vi "UndoEngine.vi"(0 "Reference In":refnum<class "Graph.lvclass">, 1 "Action":enum16{"TakeSnapshot", "Undo", "Redo"}(ring), 2 "Reset":bool, 3 "graphics":refnum<class "Graphics.lvclass">, 4 "grid":refnum<class "Grid.lvclass">, 5 "error in (no error)":errorcluster, 6 "menu":refnum<k9>, 8 "UndoLevels(ignoredIfNotWired)":i32=-1) -> (14 "Reference Out":refnum<class "Graph.lvclass">, 19 "error out":errorcluster)   [LabVIEW 2020, in "Graph.lvclass"]
doc: "Save to File"
uses:
  <resource>/Framework/Providers/Open_GDS/UML/Graph_class/Graph.lvclass
  <resource>/Framework/Providers/Open_GDS/UML/Grid_class/Grid.lvclass
  <resource>/Framework/Providers/Open_GDS/UML/Graphics_class/Graphics.lvclass
  <resource>/Framework/Providers/Open_GDS/UML/UMLEditor/UMLEditor_DiagramType.ctl
  <resource>/Framework/Providers/Open_GDS/UML/AbstractNode_class/AbstractNode.lvclass
  <resource>/Framework/Providers/Open_GDS/UML/AbstractEdge_class/AbstractEdge.lvclass
  <resource>/Framework/Providers/Open_GDS/UML/General/Rectangle/Rectangle Rectangle2D.ctl
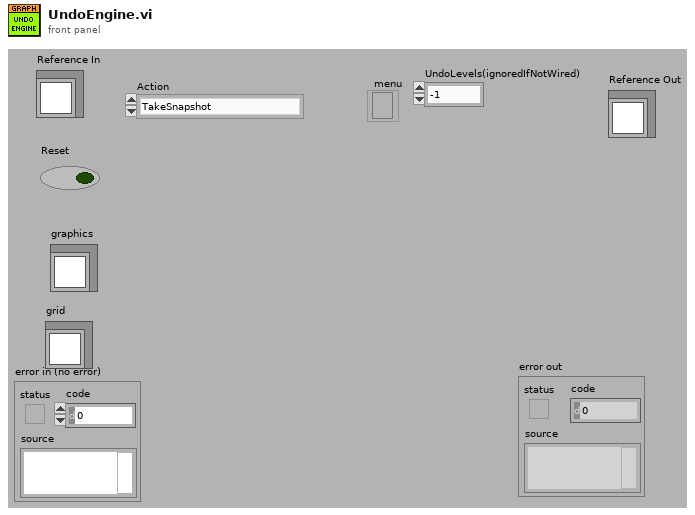
[diagram p1: front panel]
types:
  T1 = cluster{"DiagramData":string, "nodeInfo":cluster{"NodeType":string[], "ParentIndex":i32[], "ChildernIndexies":cluster{i32[]}[], "FlattenData":string[]}, "edgeInfo":cluster{"EdgeType":string[], "StartNodeIndex":i32[], "EndNodeIndex":i32[], "FlattenData":string[]}}
  T2 = cluster{"nodeInfo":cluster{"NodeType":string[], "ParentIndex":i32[], "ChildernIndexies":cluster{i32[]}[], "FlattenData":string[]}, "edgeInfo":cluster{"EdgeType":string[], "StartNodeIndex":i32[], "EndNodeIndex":i32[], "FlattenData":string[]}, "Succeeded":bool, "DiagramData":string}
  T3 = typedef "UMLEditor_DiagramType.ctl" = string
  T4 = typedef "Rectangle Rectangle2D.ctl" = cluster{"x":dbl, "y":dbl, "width":dbl, "height":dbl}
  T5 = cluster{"graph":refnum<class "Graph.lvclass">, "succeeded":bool, "diagramType":T3, "nodeInfo":cluster{"NodeType":string[], "ParentIndex":i32[], "ChildernIndexies":cluster{i32[]}[], "FlattenData":string[]}, "edgeInfo":cluster{"EdgeType":string[], "StartNodeIndex":i32[], "EndNodeIndex":i32[], "FlattenData":string[]}, "nodes":refnum<class "AbstractNode.lvclass">[], "edges":refnum<class "AbstractEdge.lvclass">[], "DiagramData":string, "bounds":T4}
  T6 = cluster{"DiagramData":string, "nodeInfo":cluster{"NodeType":string[], "ParentIndex":i32[], "ChildernIndexies":cluster{i32[]}[], "FlattenData":string[]}, "edgeInfo":cluster{"EdgeType":string[], "StartNodeIndex":i32[], "EndNodeIndex":i32[], "FlattenData":string[]}}[]
  T7 = typedef "Graph.lvclass/ObjectAttributes.ctl" = cluster{"nodes":refnum<class "AbstractNode.lvclass">[], "edges":refnum<class "AbstractEdge.lvclass">[], "nodesToBeRemoved":refnum<class "AbstractNode.lvclass">[], "edgesToBeRemoved":refnum<class "AbstractEdge.lvclass">[], "needsLayout":bool, "LayoutNodes":refnum<class "AbstractNode.lvclass">[]}
  T8 = cluster{"children":refnum<class "AbstractNode.lvclass">[]}
  T9 = cluster{"NodeType":string[], "ParentIndex":i32[], "ChildernIndexies":cluster{i32[]}[], "FlattenData":string[]}
  T10 = cluster{"EdgeType":string[], "StartNodeIndex":i32[], "EndNodeIndex":i32[], "FlattenData":string[]}
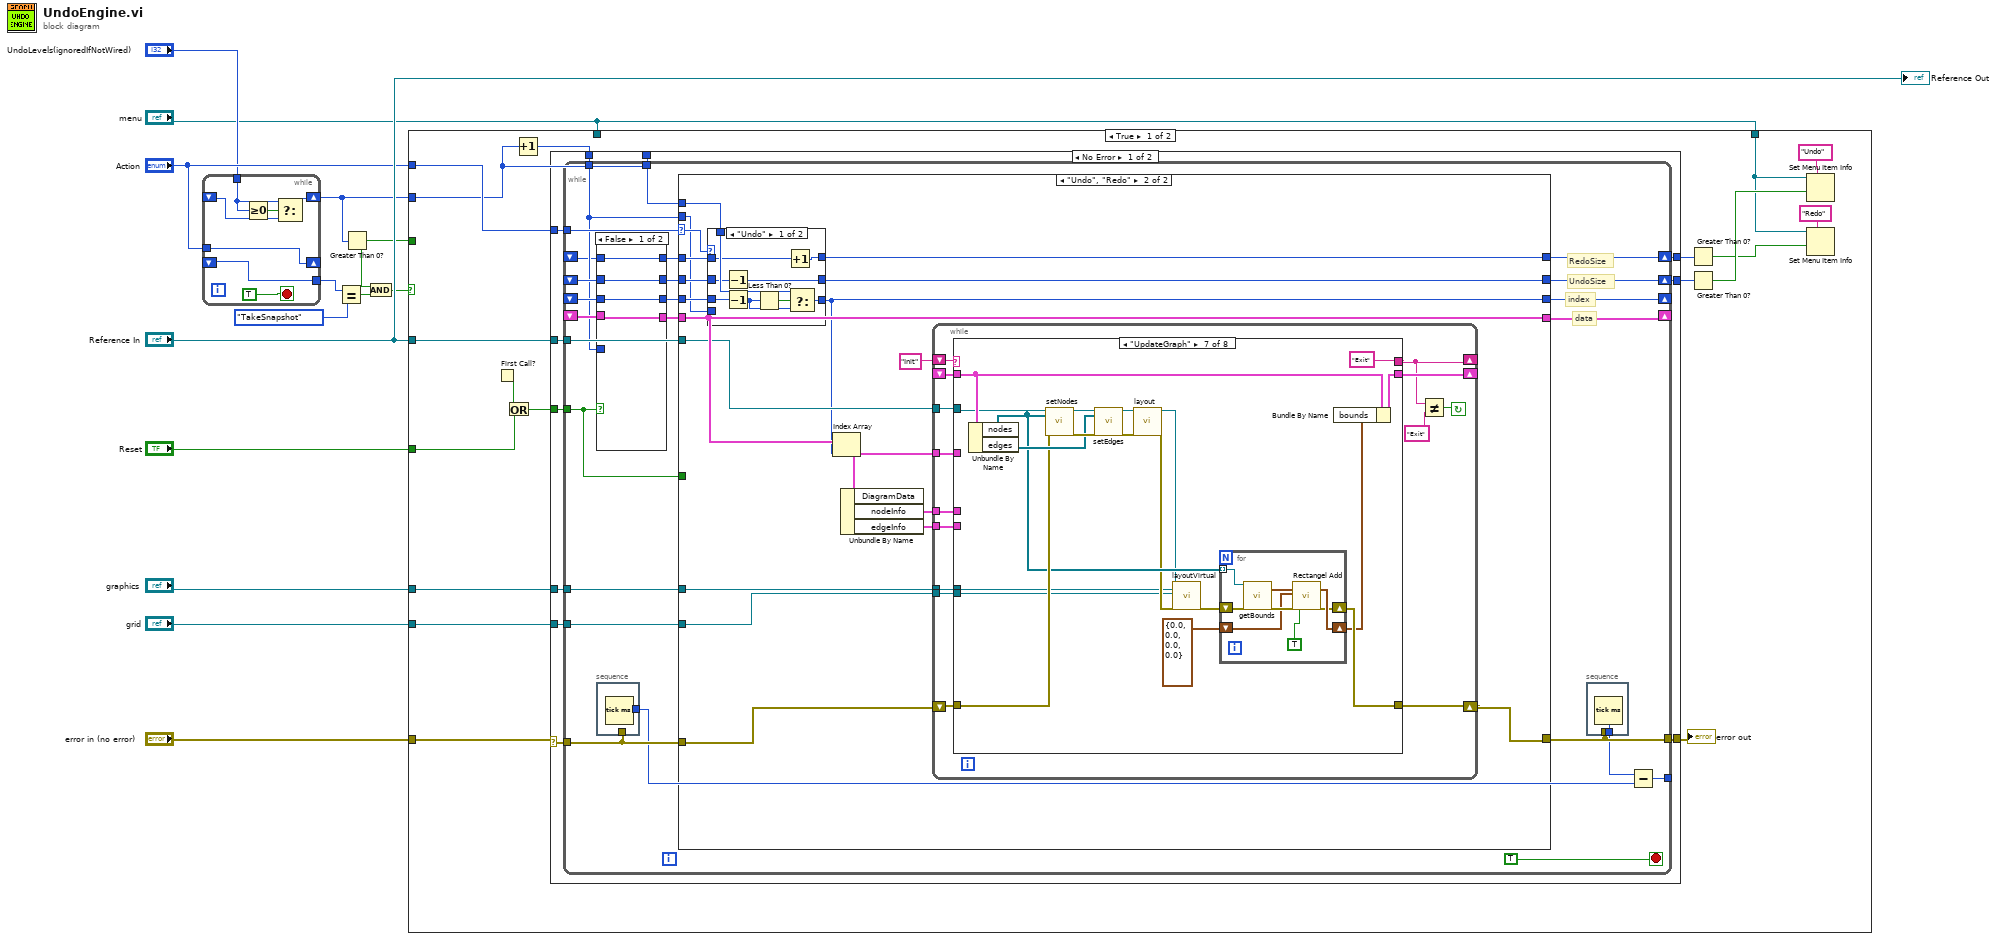
[diagram p0: block diagram]
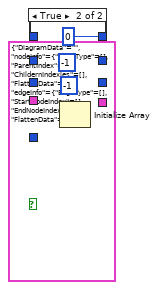
[diagram p2: hidden frame]
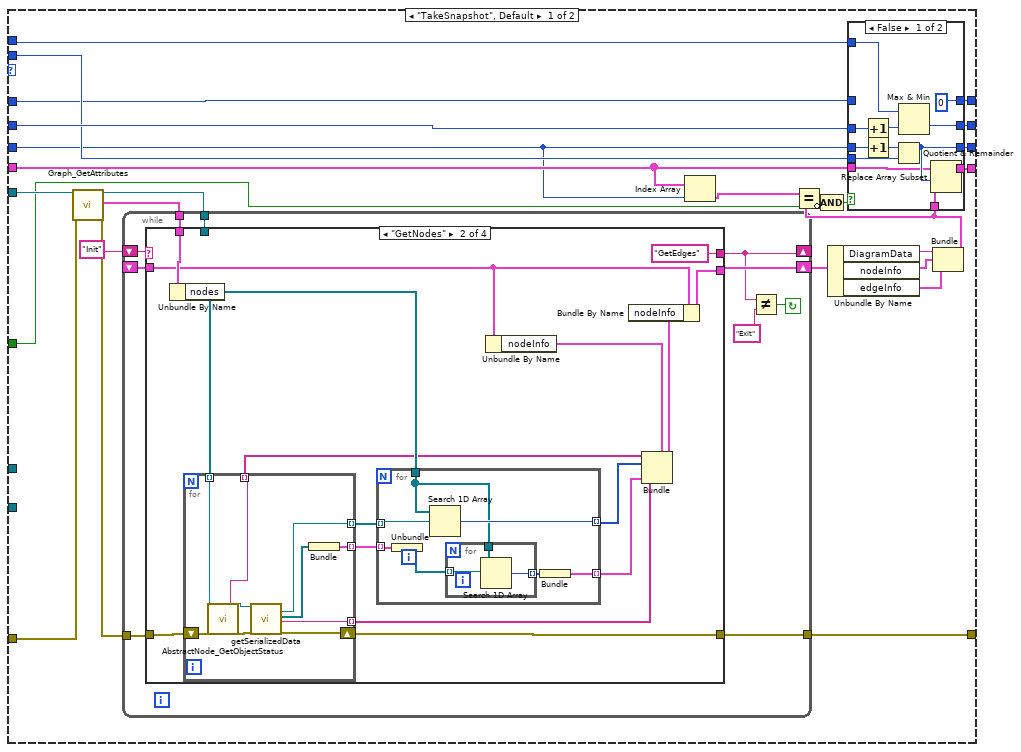
[diagram p3: hidden frame]
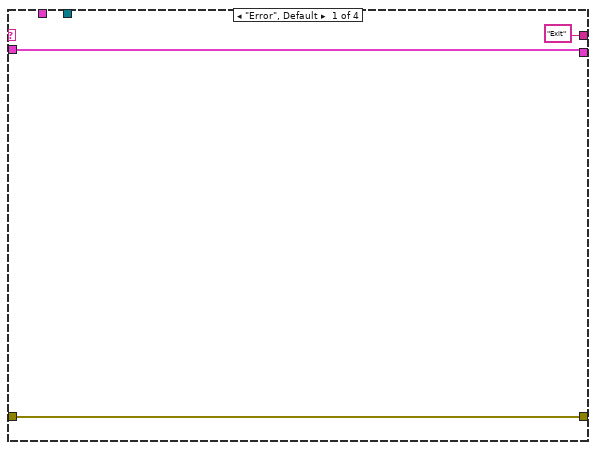
[diagram p5: hidden frame]
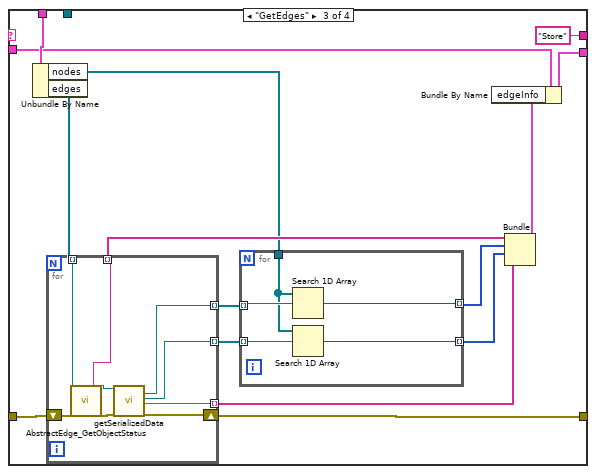
[diagram p6: hidden frame]
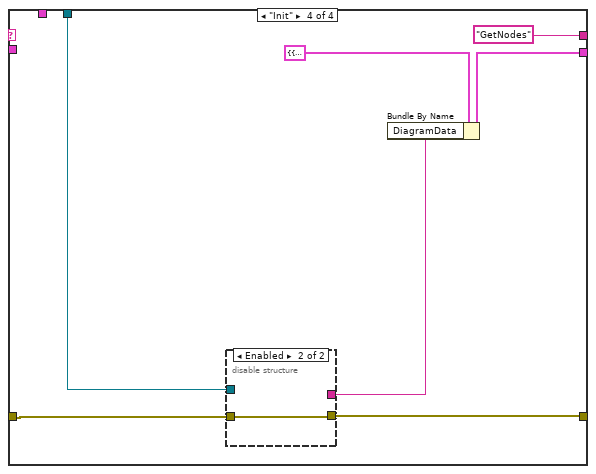
[diagram p7: hidden frame]
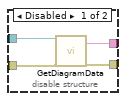
[diagram p8: hidden frame]
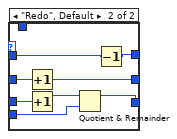
[diagram p9: hidden frame]
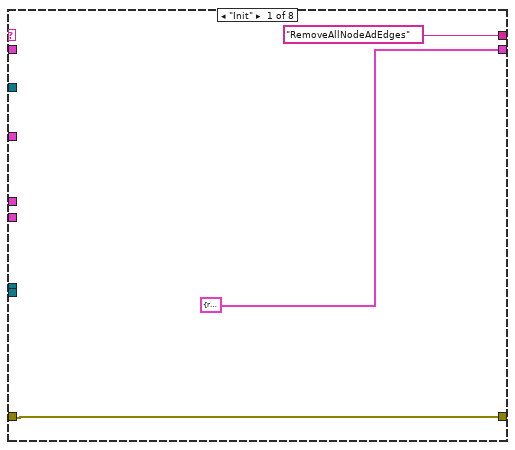
[diagram p10: hidden frame]
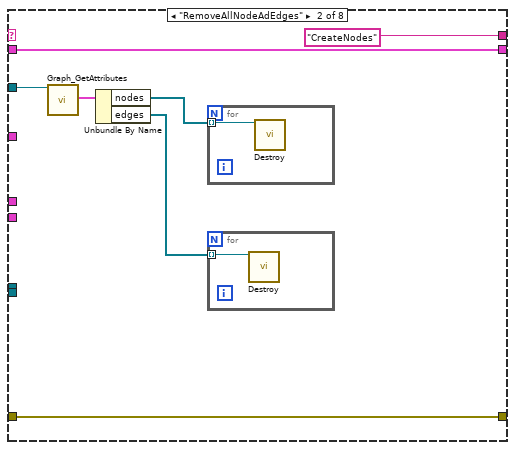
[diagram p11: hidden frame]
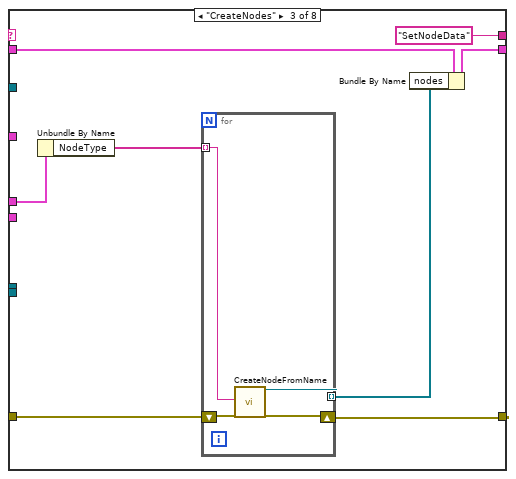
[diagram p12: hidden frame]
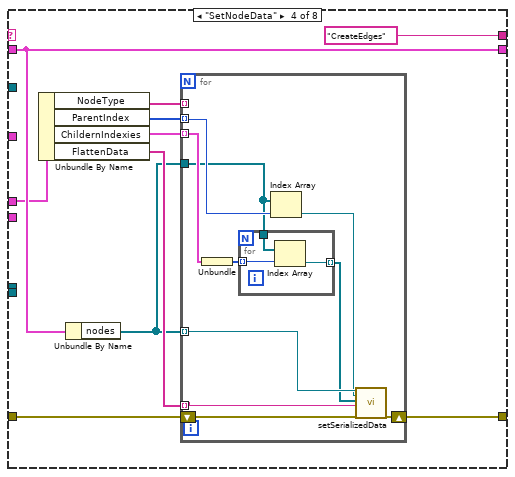
[diagram p13: hidden frame]
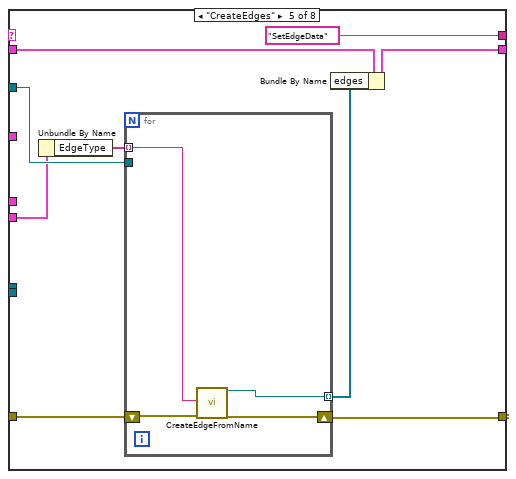
[diagram p14: hidden frame]
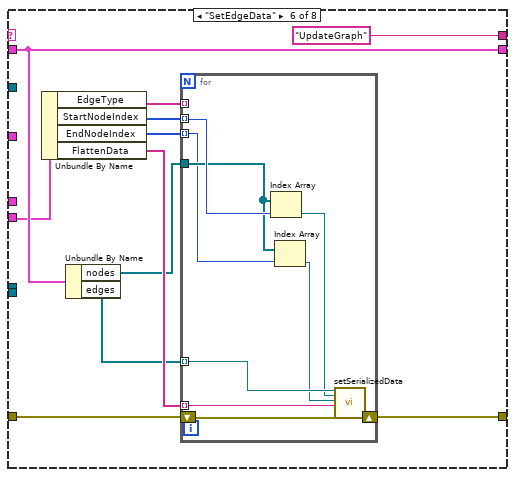
[diagram p15: hidden frame]
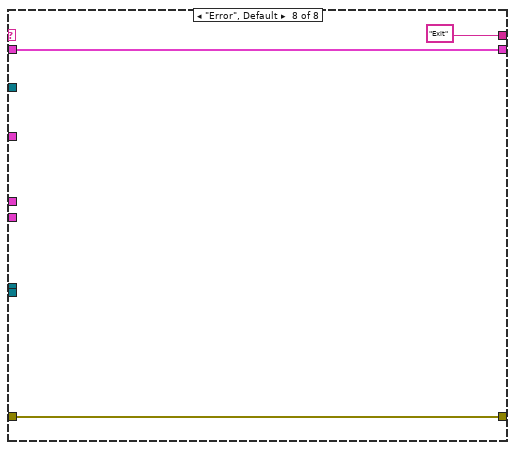
[diagram p16: hidden frame]
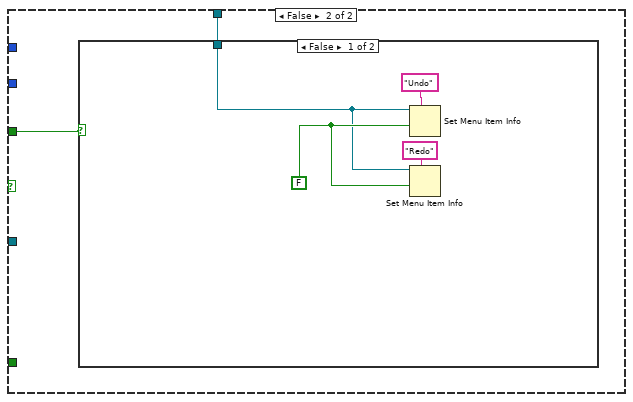
[diagram p18: hidden frame]
diagram:
  n1 = while {
    shift-right: [w19] -> _
    shift-left: _ -> [w20]
    tunnel: [w20] -> w7
    shift-right: [w15] -> w4
    shift-left: _ -> [w16]
    tunnel: "Action" -> [w19]
    tunnel: "UndoLevels(ignoredIfNotWired)" -> [w17]
    stop <- TRUE stop-if-true
    n2 = Greater Or Equal To 0?(x=w17) -> (x >= 0?=w18:bool)
    n3 = Select(t=w17, s=w18, f=w16) -> (s? t:f=w15:i32)
  }
  n4 = Equal?(x=w7, y=enum16{"TakeSnapshot", "Undo", "Redo"}."TakeSnapshot") -> (x = y?=w5:bool)
  n5 = Greater Than 0?(x=w4) -> (x > 0?=w2:bool)
  n6 = And(x=w2, y=w5) -> (x .and. y?=w3:bool)
  n7 = case shown="True" w3 {
    tunnel: "Reference In" -> [w39 _]
    tunnel: "error in (no error)" -> [w37 _]
    tunnel: "Reset" -> [w36 _]
    tunnel: "graphics" -> [w33 _]
    tunnel: "grid" -> [w32 _]
    tunnel: "Action" -> [w31 _]
    tunnel: w4 -> [w29 _]
    tunnel: w2 -> [_ w379]
    tunnel: "menu" -> [_ w378]
    tunnel: "menu" -> [w24 _]
    frame True {
      n8 = First Call?() -> (First Call?: T/F=w35:bool)
      n9 = Or(x=w35, y=w36) -> (x .or. y?=w34:bool)
      n10 = Increment(x=w29) -> (x+1=w30:i32)
      n11 = case shown="No Error" w37 {
        selector: w37 -> [w48 w377]
        tunnel: w39 -> [w50 _]
        tunnel: [w49 w377] -> w38
        tunnel: w31 -> [w47 _]
        tunnel: w34 -> [w46 _]
        tunnel: [w45 _] -> w22
        tunnel: w30 -> [w44 _]
        tunnel: w33 -> [w43 _]
        tunnel: w32 -> [w42 _]
        tunnel: w29 -> [w41 _]
        tunnel: [w40 _] -> w23
        frame No Error {
          n12 = while {
            tunnel: w50 -> [w75]
            tunnel: [w55] -> w49
            tunnel: w48 -> [w54]
            tunnel: w47 -> [w74]
            shift-right: [w64] -> _
            shift-left: _ -> [w69]
            shift-right: [w70] -> _
            shift-left: _ -> [w72]
            tunnel: w46 -> [w61]
            shift-right: [w65] -> w45
            shift-left: _ -> [w67]
            tunnel: w44 -> [w60]
            tunnel: w43 -> [w63]
            tunnel: w42 -> [w62]
            tunnel: w41 -> [w59]
            shift-right: [w56] -> w40
            shift-left: _ -> [w58]
            tunnel: [w51] -> _
            stop <- TRUE stop-if-true
            # "RedoSize"
            # "data"
            # "UndoSize"
            # "index"
            n13 = case shown="False" w61 {
              tunnel: w72 -> [w80 _]
              tunnel: [w80 -1] -> w71
              tunnel: w69 -> [w79 _]
              tunnel: [w79 w85] -> w68
              tunnel: w67 -> [w81 _]
              tunnel: [w81 -1] -> w66
              tunnel: w60 -> [_ w83]
              tunnel: [w78 0] -> w57
              tunnel: w58 -> [w78 _]
              frame False {
              }
              frame True {
                n14 = Initialize Array(T1 {"DiagramData"="", "nodeInfo"={"NodeType"=[], "ParentIndex"=[], "ChildernIndexies"=[], "FlattenData"=[]}, "edgeInfo"={"EdgeType"=[], "StartNodeIndex"=[], "EndNodeIndex"=[], "FlattenData"=[]}} ("output cluster"), w83) -> (w85:T6)
              }
            }
            n15 = stacked-sequence {
              tunnel: w54 -> [_]
              tunnel: [w76] -> w52
              frame #0 {
                n16 = Tick Count (ms)() -> (millisecond timer value=w76:u32)
              }
            }
            n17 = case shown="\"Undo\", \"Redo\"" w74 {
              selector: w74 -> [_ w224]
              tunnel: w75 -> [w113 w232]
              tunnel: [w112 w230] -> w55
              tunnel: w54 -> [w89 w231]
              tunnel: w71 -> [w98 w235]
              tunnel: [w102 w227] -> w70
              tunnel: w68 -> [w99 w233]
              tunnel: w66 -> [w104 w226]
              tunnel: [w100 w234] -> w65
              tunnel: w60 -> [w101 w218]
              tunnel: [w103 w233] -> w64
              tunnel: w63 -> [_ w229]
              tunnel: w62 -> [_ w228]
              tunnel: w61 -> [w93 _]
              tunnel: w59 -> [w91 w217]
              tunnel: w57 -> [w90 w223]
              tunnel: [w92 w225] -> w56
              frame "TakeSnapshot", Default {
                n18 = call <resource>:"Graph_GetAttributes.vi"("reference in"=w113, "error in (no error)"=w89) -> ("reference out"=w111:refnum<class "Graph.lvclass">, "Data"=w88:T7, "error out"=w110:errorcluster)  [unwired: 1 in, 14 out]
                n19 = while {
                  tunnel: w88 -> [w139]
                  tunnel: w110 -> [w138]
                  tunnel: [w137] -> w112
                  shift-right: [w132] -> _
                  shift-left: "Init" -> [w136]
                  shift-right: [w135] -> w108
                  shift-left: _ -> [w131]
                  tunnel: w111 -> [w130]
                  stop <- w133 continue-if-true
                  n20 = case shown="\"GetNodes\"" w136 {
                    tunnel: w139 -> [_ w157 w191 _]
                    tunnel: w138 -> [w142 w156 w190 w208]
                    tunnel: [w142 w150 w177 w207] -> w137
                    tunnel: [w140 w146 w183 w209] -> w135
                    tunnel: ["Exit" ("y") "GetEdges" "Store" "GetNodes"] -> w132
                    tunnel: w131 -> [w140 w144 w185 _]
                    tunnel: w130 -> [_ _ _ w205]
                    frame "Error", Default {
                    }
                    frame "GetNodes" {
                      n21 = Unbundle By Name(w157) -> ("nodes"=w149:refnum<class "AbstractNode.lvclass">[])
                      n22 = for {
                        shift-right: [w169] -> w150
                        shift-left: w156 -> [w176]
                        tunnel: w149 -> [w172] mode=indexing
                        tunnel: [w175] -> w155 mode=indexing
                        tunnel: [w173] -> w154 mode=indexing
                        tunnel: [w170] -> w151 mode=indexing
                        tunnel: [w168] -> w148 mode=indexing
                        n23 = call <resource>:"AbstractNode_GetObjectStatus.vi"("reference in"=w172) -> ("Class name"=w168:string, "reference out"=w171:refnum<class "AbstractNode.lvclass">)  [unwired: 1 in, 16 out]
                        n24 = call-dynamic "getSerializedData.vi"("reference"=w171, "error in (no error)"=w176) -> ("parent"=w175:refnum<class "AbstractNode.lvclass">, "children"=w174:refnum<class "AbstractNode.lvclass">[], "xmlOut"=w170:string, "error out"=w169:errorcluster)  [unwired: 13 in, 1 out]
                        n25 = Bundle("children"=w174) -> (w173:T8)  [unwired: 1 in]
                      }
                      n26 = for {
                        tunnel: w155 -> [w163] mode=indexing
                        tunnel: w154 -> [w164] mode=indexing
                        tunnel: [w162] -> w153 mode=indexing
                        tunnel: [w159] -> w152 mode=indexing
                        tunnel: w149 -> [w158]
                        n27 = Unbundle(w164) -> ("children"=w161:refnum<class "AbstractNode.lvclass">[])
                        n28 = Search 1D Array(1D array=w158, element=w163) -> (index of element=w162:i32)  [unwired: 1 out]
                        n29 = for {
                          tunnel: w161 -> [w166] mode=indexing
                          tunnel: w158 -> [w167]
                          tunnel: [w165] -> w160 mode=indexing
                          n30 = Search 1D Array(1D array=w167, element=w166) -> (index of element=w165:i32)  [unwired: 1 out]
                        }
                        n31 = Bundle(w160) -> (w159:cluster{i32[]})  [unwired: 1 in]
                      }
                      n32 = Unbundle By Name(w144) -> ("nodeInfo"=w143:T9)
                      n33 = Bundle(cluster=w143, "NodeType"=w148, "ParentIndex"=w153, "ChildernIndexies"=w152, "FlattenData"=w151) -> (w147:T9)
                      n34 = Bundle By Name(cluster=w144, "nodeInfo"=w147) -> (w146:T2)
                    }
                    frame "GetEdges" {
                      n35 = Unbundle By Name(w191) -> ("nodes"=w181:refnum<class "AbstractNode.lvclass">[], "edges"=w180:refnum<class "AbstractEdge.lvclass">[])
                      n36 = for {
                        shift-right: [w198] -> w177
                        shift-left: w190 -> [w204]
                        tunnel: w180 -> [w202] mode=indexing
                        tunnel: [w203] -> w189 mode=indexing
                        tunnel: [w199] -> w187 mode=indexing
                        tunnel: [w197] -> w186 mode=indexing
                        tunnel: [w200] -> w179 mode=indexing
                        n37 = call <resource>:"AbstractEdge_GetObjectStatus.vi"("reference in"=w202) -> ("Class name"=w197:string, "reference out"=w201:refnum<class "AbstractEdge.lvclass">)  [unwired: 1 in, 16 out]
                        n38 = call-dynamic "getSerializedData.vi"("reference"=w201, "error in (no error)"=w204) -> ("startNode"=w203:refnum<class "AbstractNode.lvclass">, "endNode"=w200:refnum<class "AbstractNode.lvclass">, "xmlOut"=w199:string, "error out"=w198:errorcluster)  [unwired: 13 in, 1 out]
                      }
                      n39 = for {
                        tunnel: w189 -> [w196] mode=indexing
                        tunnel: [w195] -> w188 mode=indexing
                        tunnel: w181 -> [w194]
                        tunnel: w179 -> [w193] mode=indexing
                        tunnel: [w192] -> w178 mode=indexing
                        n40 = Search 1D Array(1D array=w194, element=w196) -> (index of element=w195:i32)  [unwired: 1 out]
                        n41 = Search 1D Array(1D array=w194, element=w193) -> (index of element=w192:i32)  [unwired: 1 out]
                      }
                      n42 = Bundle(w186, w188, w178, w187) -> (w184:cluster{string[], i32[], i32[], string[]})  [unwired: 1 out]
                      n43 = Bundle By Name(cluster=w185, "edgeInfo"=w184) -> (w183:T2)
                    }
                    frame "Init" {
                      n44 = disable-structure shown="Enabled" {
                        disable-tunnel: w208 -> [w215 w216]
                        disable-tunnel: [w214 w216] -> w207
                        disable-tunnel: [w213 _] -> w206
                        disable-tunnel: w205 -> [w212 _]
                        frame Disabled {
                          n45 = call-dynamic "GetDiagramData.vi"("reference"=w212, "error in (no error)"=w215) -> ("DiagramData"=w213:string, "error out"=w214:errorcluster)  [unwired: 15 in, 1 out]
                        }
                        frame Enabled {
                        }
                      }
                      n46 = Bundle By Name(cluster=T2 {"nodeInfo"={"NodeType"=[], "ParentIndex"=[], "ChildernIndexies"=[], "FlattenData"=[]}, "edgeInfo"={"EdgeType"=[], "StartNodeIndex"=[], "EndNodeIndex"=[], "FlattenData"=[]}, "Succeeded"=FALSE, "DiagramData"=""}, "DiagramData"=w206) -> (w209:T2)
                    }
                  }
                  n47 = Not Equal?(x=w132, y="Exit") -> (x != y?=w133:bool)
                }
                n48 = Index Array(array=w99, index=w98) -> (element=w96:T1)
                n49 = Unbundle By Name(w108) -> ("DiagramData"=w107:string, "nodeInfo"=w106:T9, "edgeInfo"=w105:T10)
                n50 = Bundle("DiagramData"=w107, "nodeInfo"=w106, "edgeInfo"=w105) -> (w97:T1)  [unwired: 1 out]
                n51 = Equal?(x=w96, y=w97) -> (x = y?=w95:bool)
                n52 = Compound Arithmetic op=AND(w95, invert w93) -> (w94:bool)
                n53 = case shown="False" w94 {
                  tunnel: w104 -> [w125 w129]
                  tunnel: [w123 w127] -> w103
                  tunnel: [w122 w128] -> w102
                  tunnel: w101 -> [w115 _]
                  tunnel: [w120 w129] -> w100
                  tunnel: w99 -> [w119 w127]
                  tunnel: w98 -> [w118 w128]
                  tunnel: w97 -> [w117 _]
                  tunnel: w91 -> [w116 _]
                  tunnel: [0 w126] -> w92
                  tunnel: w90 -> [_ w126]
                  frame False {
                    n54 = Increment(x=w125) -> (x+1=w121:i32)
                    n55 = Increment(x=w118) -> (x+1=w124:i32)
                    n56 = Quotient & Remainder(x=w124, y=w115) -> (x-y*floor(x/y)=w122:i32)  [unwired: 1 out]
                    n57 = Max & Min(x=w116, y=w121) -> (min(x,y)=w120:i32)  [unwired: 1 out]
                    n58 = Replace Array Subset(array=w119, new element=w117, index=w122) -> (w123:T6)
                  }
                  frame True {
                  }
                }
              }
              frame "Undo", "Redo" {
                n59 = case shown="\"Undo\"" w224 {
                  tunnel: w235 -> [w244 w252]
                  tunnel: [w243 w251] -> w234
                  tunnel: w217 -> [w240 _]
                  tunnel: [w239 w246] -> w227
                  tunnel: w226 -> [w238 w250]
                  tunnel: w223 -> [w237 w249]
                  tunnel: [w236 w248] -> w225
                  tunnel: w218 -> [_ w245]
                  frame "Undo" {
                    n60 = Decrement(x=w238) -> (x-1=w243:i32)
                    n61 = Decrement(x=w244) -> (x-1=w241:i32)
                    n62 = Less Than 0?(x=w241) -> (x < 0?=w242:bool)
                    n63 = Increment(x=w237) -> (x+1=w236:i32)
                    n64 = Select(t=w240, s=w242, f=w241) -> (s? t:f=w239:i32)
                  }
                  frame "Redo", Default {
                    n65 = Increment(x=w250) -> (x+1=w251:i32)
                    n66 = Increment(x=w252) -> (x+1=w247:i32)
                    n67 = Quotient & Remainder(x=w247, y=w245) -> (x-y*floor(x/y)=w246:i32)  [unwired: 1 out]
                    n68 = Decrement(x=w249) -> (x-1=w248:i32)
                  }
                }
                n69 = Index Array(array=w233, index=w227) -> (element=w221:T1)
                n70 = Unbundle By Name(w221) -> ("nodeInfo"=w220:T9, "edgeInfo"=w219:T10)  [unwired: 1 out]
                n71 = while {
                  shift-right: [w262] -> _
                  shift-left: "Init" -> [w266]
                  shift-right: [w265] -> _
                  shift-left: _ -> [w261]
                  shift-right: [w259] -> w230
                  shift-left: w231 -> [w260]
                  tunnel: w229 -> [w258]
                  tunnel: w228 -> [w257]
                  tunnel: w221 -> [w256]
                  tunnel: w232 -> [w255]
                  tunnel: w220 -> [w254]
                  tunnel: w219 -> [w253]
                  stop <- w263 continue-if-true
                  n72 = case shown="\"UpdateGraph\"" w266 {
                    tunnel: w260 -> [w269 w276 w284 w295 w320 w332 w360 w376]
                    tunnel: [w269 w276 w280 w294 w317 w331 w355 w376] -> w259
                    tunnel: [T5 {"graph"=refnum, "succeeded"=FALSE, "diagramType"="", "nodeInfo"={"NodeType"=[], "ParentIndex"=[], "ChildernIndexies"=[], "FlattenData"=[]}, "edgeInfo"={"EdgeType"=[], "StartNodeIndex"=[], "EndNodeIndex"=[], "FlattenData"=[]}, "nodes"=[], "edges"=[], "DiagramData"="", "bounds"={"x"=0.0, "y"=0.0, "width"=0.0, "height"=0.0}} ("localData") w272 w282 w293 w319 w330 w358 w374] -> w265
                    tunnel: ["RemoveAllNodeAdEdges" "CreateNodes" "SetNodeData" "CreateEdges" ("y") "SetEdgeData" "UpdateGraph" ("y") "Exit" ("y") "Exit" ("y")] -> w262
                    tunnel: w261 -> [_ w272 w281 w293 w318 w330 w357 w374]
                    tunnel: w258 -> [_ _ _ _ _ _ w349 _]
                    tunnel: w257 -> [_ _ _ _ _ _ w348 _]
                    tunnel: w256 -> [_ _ _ _ _ _ _ _]
                    tunnel: w255 -> [_ w275 _ _ w315 _ w347 _]
                    tunnel: w254 -> [_ _ w279 w291 _ _ _ _]
                    tunnel: w253 -> [_ _ _ _ w314 w327 _ _]
                    frame "Init" {
                    }
                    frame "RemoveAllNodeAdEdges" {
                      n73 = call <resource>:"Graph_GetAttributes.vi"("reference in"=w275) -> ("Data"=w270:T7)  [unwired: 2 in, 16 out]
                      n74 = Unbundle By Name(w270) -> ("nodes"=w274:refnum<class "AbstractNode.lvclass">[], "edges"=w273:refnum<class "AbstractEdge.lvclass">[])
                      n75 = for {
                        tunnel: w274 -> [w278] mode=indexing
                        n76 = call-dynamic "Destroy.vi"("reference"=w278) -> ()  [unwired: 17 in, 2 out]
                      }
                      n77 = for {
                        tunnel: w273 -> [w277] mode=indexing
                        n78 = call-dynamic "Destroy.vi"("reference"=w277) -> ()  [unwired: 18 in, 1 out]
                      }
                    }
                    frame "CreateNodes" {
                      n79 = Unbundle By Name(w279) -> ("NodeType"=w285:string[])
                      n80 = for {
                        tunnel: w285 -> [w289] mode=indexing
                        shift-right: [w288] -> w280
                        shift-left: w284 -> [w290]
                        tunnel: [w287] -> w283 mode=indexing
                        n81 = call <resource>:"CreateNodeFromName.vi"("NodeTypeToCreate"=w289, "error in (no error)"=w290) -> ("NodeCreated"=w287:refnum<class "AbstractNode.lvclass">, "error out"=w288:errorcluster)  [unwired: 16 in]
                      }
                      n82 = Bundle By Name(cluster=w281, "nodes"=w283) -> (w282:T5)
                    }
                    frame "SetNodeData" {
                      n83 = Unbundle By Name(w291) -> ("NodeType"=w299:string[], "ParentIndex"=w298:i32[], "ChildernIndexies"=w297:cluster{i32[]}[], "FlattenData"=w296:string[])
                      n84 = Unbundle By Name(w293) -> ("nodes"=w292:refnum<class "AbstractNode.lvclass">[])
                      n85 = for {
                        tunnel: w299 -> [_] mode=indexing
                        tunnel: w298 -> [w310] mode=indexing
                        tunnel: w297 -> [w309] mode=indexing
                        tunnel: w292 -> [w308]
                        tunnel: w292 -> [w306] mode=indexing
                        tunnel: w296 -> [w302] mode=indexing
                        shift-right: [w303] -> w294
                        shift-left: w295 -> [w301]
                        n86 = Unbundle(w309) -> (w307:i32[])
                        n87 = for {
                          tunnel: w308 -> [w313]
                          tunnel: w307 -> [w312] mode=indexing
                          tunnel: [w311] -> w304 mode=indexing
                          n88 = Index Array(array=w313, index=w312) -> (element=w311:refnum<class "AbstractNode.lvclass">)
                        }
                        n89 = Index Array(array=w308, index=w310) -> (element=w305:refnum<class "AbstractNode.lvclass">)
                        n90 = call-dynamic "setSerializedData.vi"("reference"=w306, "parent"=w305, "children"=w304, "xmlOut"=w302, "error in (no error)"=w301) -> ("error out"=w303:errorcluster)  [unwired: 13 in, 1 out]
                      }
                    }
                    frame "CreateEdges" {
                      n91 = Unbundle By Name(w314) -> ("EdgeType"=w321:string[])
                      n92 = for {
                        tunnel: w321 -> [w324] mode=indexing
                        shift-right: [w325] -> w317
                        shift-left: w320 -> [w326]
                        tunnel: w315 -> [_]
                        tunnel: [w323] -> w316 mode=indexing
                        n93 = call <resource>:"CreateEdgeFromName.vi"("NodeTypeToCreate"=w324, "error in (no error)"=w326) -> ("AbstractCreated"=w323:refnum<class "AbstractEdge.lvclass">, "error out"=w325:errorcluster)  [unwired: 16 in]
                      }
                      n94 = Bundle By Name(cluster=w318, "edges"=w316) -> (w319:T5)
                    }
                    frame "SetEdgeData" {
                      n95 = Unbundle By Name(w327) -> ("EdgeType"=w336:string[], "StartNodeIndex"=w335:i32[], "EndNodeIndex"=w334:i32[], "FlattenData"=w333:string[])
                      n96 = Unbundle By Name(w330) -> ("nodes"=w329:refnum<class "AbstractNode.lvclass">[], "edges"=w328:refnum<class "AbstractEdge.lvclass">[])
                      n97 = for {
                        tunnel: w336 -> [_] mode=indexing
                        tunnel: w335 -> [w346] mode=indexing
                        tunnel: w334 -> [w340] mode=indexing
                        tunnel: w329 -> [w345]
                        tunnel: w328 -> [w344] mode=indexing
                        tunnel: w333 -> [w339] mode=indexing
                        shift-right: [w341] -> w331
                        shift-left: w332 -> [w338]
                        n98 = Index Array(array=w345, index=w346) -> (element=w343:refnum<class "AbstractNode.lvclass">)
                        n99 = Index Array(array=w345, index=w340) -> (element=w342:refnum<class "AbstractNode.lvclass">)
                        n100 = call-dynamic "setSerializedData.vi"("reference"=w344, "startNode"=w343, "endNode"=w342, "xmlOut"=w339, "error in (no error)"=w338) -> ("error out"=w341:errorcluster)  [unwired: 13 in, 1 out]
                      }
                    }
                    frame "UpdateGraph" {
                      n101 = Unbundle By Name(w357) -> ("nodes"=w354:refnum<class "AbstractNode.lvclass">[], "edges"=w363:refnum<class "AbstractEdge.lvclass">[])
                      n102 = call-dynamic "setNodes.vi"("reference"=w347, "nodes"=w354, "error in (no error)"=w360) -> ("reference out"=w365:refnum<class "Graph.lvclass">, "error out"=w364:errorcluster)  [unwired: 15 in]
                      n103 = call-dynamic "setEdges.vi"("reference"=w365, "edges"=w363, "error in (no error)"=w364) -> ("reference out"=w362:refnum<class "Graph.lvclass">, "error out"=w361:errorcluster)  [unwired: 15 in]
                      n104 = call-dynamic "layout.vi"("reference"=w362, "error in (no error)"=w361) -> ("reference out"=w351:refnum<class "Graph.lvclass">, "error out"=w350:errorcluster)  [unwired: 16 in]
                      n105 = call <resource>:"layoutVirtual.vi"("reference"=w351, "graphics"=w349, "grid"=w348, "error in (no error)"=w350) -> ("error out"=w352:errorcluster)  [unwired: 15 out]
                      n106 = for {
                        shift-right: [w368] -> w355
                        shift-left: w352 -> [w367]
                        shift-right: [w369] -> w353
                        shift-left: T4 {"x"=0.0, "y"=0.0, "width"=0.0, "height"=0.0} ("boundsAdded") -> [w370]
                        tunnel: w354 -> [w366] mode=indexing
                        n107 = call-dynamic "getBounds.vi"("reference"=w366, "error in (no error)"=w367) -> ("bounds"=w373:T4, "error out"=w372:errorcluster)  [unwired: 15 in, 1 out]
                        n108 = call <resource>:"Rectangel Add.vi"("bounds1"=w373, "bounds2"=w370, "error in (no error)"=w372, "useAbsoluteCordinates(False)"=TRUE) -> ("boundsAdded"=w369:T4, "error out"=w368:errorcluster)  [unwired: 1 in, 13 out]
                      }
                      n109 = Bundle By Name(cluster=w357, "bounds"=w353) -> (w358:T5)
                    }
                    frame "Error", Default {
                    }
                  }
                  n110 = Not Equal?(x=w262, y="Exit") -> (x != y?=w263:bool)
                }
              }
            }
            n111 = stacked-sequence {
              tunnel: w55 -> [_]
              tunnel: [w77] -> w53
              frame #0 {
                n112 = Tick Count (ms)() -> (millisecond timer value=w77:u32)
              }
            }
            n113 = Subtract(x=w53, y=w52) -> (x-y=w51:u32)
          }
        }
        frame Error {
        }
      }
      "error out" <- w38
      n114 = Greater Than 0?(x=w23) -> (x > 0?=w25:bool)
      n115 = Greater Than 0?(x=w22) -> (x > 0?=w27:bool)
      n116 = Set Menu Item Info(7:"Undo" ("item tag"), 9:w27, 11:w24) -> ()  [unwired: 1 in, 5 out]
      n117 = Set Menu Item Info(7:"Redo" ("item tag"), 9:w25, 11:w24) -> ()  [unwired: 1 in, 5 out]
    }
    frame False {
      n118 = case shown="False" w379 {
        tunnel: w378 -> [w380 _]
        frame False {
          w381 = FALSE
          n119 = Set Menu Item Info(7:"Undo" ("item tag"), 9:w381, 11:w380) -> ()  [unwired: 1 in, 5 out]
          n120 = Set Menu Item Info(7:"Redo" ("item tag"), 9:w381, 11:w380) -> ()  [unwired: 1 in, 5 out]
        }
        frame True {
        }
      }
    }
  }
  "Reference Out" <- "Reference In"
